vi "Write Raw.vi"(8 "error in (no error)":errorcluster, 10 "Data In":u8[](array[numeric]) format="%.0x", 11 "Writer Reference":T1 {"refnum" format="%.0x"}) -> (0 "error out":errorcluster, 2 "Data Out":u8[](array[numeric]) format="%.0x")   [LabVIEW 2021, in "Iceoryx.lvlib"]
doc: "Raw writer does not support variable size data and must always write the full array. It is 2x as effecient as it removes a mem copy."
uses:
  Iceoryx.lvlib
  Refnum/Typedef/BB Raw Writer Refnum.ctl
  SubVIs/Convert Error Core.vi
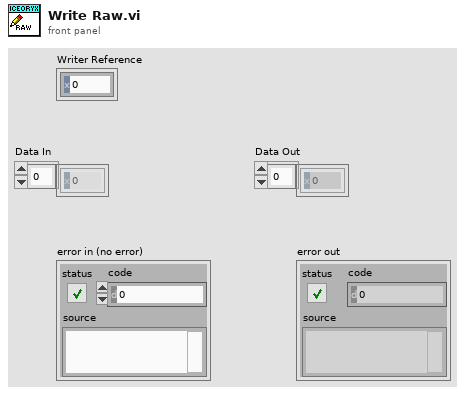
[diagram p1: front panel]
types:
  T1 = typedef "Iceoryx.lvlib/BB Raw Writer Refnum.ctl" = cluster{"refnum":u64, "BB Raw Writer":enum8{"bb_raw_writer"}}
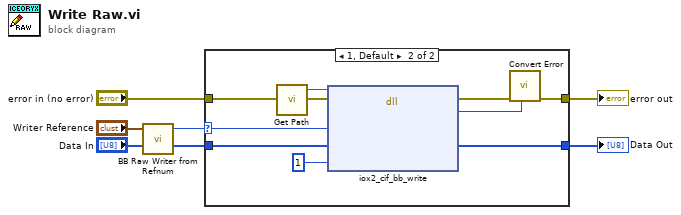
[diagram p0: block diagram]
diagram:
  n1 = call "BB Raw Writer from Refnum.vi"("BB Raw Writer Refnum"="Writer Reference") -> ("BB Raw Writer U64"=w3:u64)  [unwired: 4 in]
  n2 = case shown="1, Default" w3 {
    selector: w3 -> [_ w11]
    tunnel: "error in (no error)" -> [w8 w17]
    tunnel: "Data In" -> [w7 w10]
    tunnel: [w7 w15] -> w1
    tunnel: [w8 w12] -> w5
    frame 0 {
    }
    frame 1, Default {
      n3 = call "Get Path.vi"() -> ("libiox2_cif path"=w16:path)  [unwired: 4 in]
      n4 = dll-call lib="D:/dev/iceoryx2_lvwrapper/dist/iox2_cif.dll" fn="iox2_cif_bb_write"(path in=w16, error in=w17, "writer"=w11, "elems"=w10, "count"=u32 1 ("max_count")) -> (error out=w14:errorcluster, "return type"=w13:i32, "elems"=w15:u8[])  [unwired: 3 in, 1 out]
      n5 = call "Convert Error.vi"("return type"=w13, "error in (no error)"=w14) -> ("error out"=w12:errorcluster)  [unwired: 9 in]
    }
  }
  "error out" <- w5
  "Data Out" <- w1
